vi "PathPlanner_Path_PreCalcValues.vi"(11 "PathPlannerPath":T1={"Reversed"=FALSE, "RotationTargets"=[], "ConstraintZones"=[], "EventMarkers"=[], "GlobalConstraints"={"MaxVelocityMps;"=0.0, "MaxAccelerationMpsSq;"=0.0, "MaxAngularVelRadPsEc;"=0.0, "MaxAngularAccRadPSecSq"=0.0, "Exists"=FALSE, "Unlimited"=FALSE, "NominalVoltageVolts"=12.0}, "GoalEndState"={"VelocityMPS"=0.0, "Rotation"={"VALUE"=0.0, "COS"=1.0, "SIN"=0.0}}, "AllPoints"=[], "Name"="", "Waypoints"=[], "PointTowardsZones"=[], "IdealStartingState"={"VelocityMPS"=0.0, "Rotation"={"VALUE"=1.0, "COS"=0.0, "SIN"=0.0}}, "IsChoreoPath"=FALSE, "PreventFlipping"=FALSE} {"IdealStartingState"."Rotation"."SIN" format="%13.4f"; "IdealStartingState"."Rotation"."COS" format="%13.4f"; "IdealStartingState"."Rotation"."VALUE" format="%13.4f"; "PointTowardsZones"."TargetPosition"."Y" format="%14.3f"; "PointTowardsZones"."TargetPosition"."X" format="%14.3f"; "PointTowardsZones"."RotationOffset"."SIN" format="%13.4f"; "PointTowardsZones"."RotationOffset"."COS" format="%13.4f"; "PointTowardsZones"."RotationOffset"."VALUE" format="%13.4f"; "Waypoints"."nextControl"."Y" format="%14.3f"; "Waypoints"."nextControl"."X" format="%14.3f"; "Waypoints"."anchor"."Y" format="%14.3f"; "Waypoints"."anchor"."X" format="%14.3f"; "Waypoints"."prevControl"."Y" format="%14.3f"; "Waypoints"."prevControl"."X" format="%14.3f"; "AllPoints"."RotationTarget"."rotation"."SIN" format="%13.4f"; "AllPoints"."RotationTarget"."rotation"."COS" format="%13.4f"; "AllPoints"."RotationTarget"."rotation"."VALUE" format="%13.4f"; "AllPoints"."Position"."Y" format="%14.3f"; "AllPoints"."Position"."X" format="%14.3f"; "GoalEndState"."Rotation"."SIN" format="%13.4f"; "GoalEndState"."Rotation"."COS" format="%13.4f"; "GoalEndState"."Rotation"."VALUE" format="%13.4f"; "RotationTargets"."rotation"."SIN" format="%13.4f"; "RotationTargets"."rotation"."COS" format="%13.4f"; "RotationTargets"."rotation"."VALUE" format="%13.4f"}) -> (3 "out PathPlannerPath":T1={"Reversed"=FALSE, "RotationTargets"=[], "ConstraintZones"=[], "EventMarkers"=[], "GlobalConstraints"={"MaxVelocityMps;"=0.0, "MaxAccelerationMpsSq;"=0.0, "MaxAngularVelRadPsEc;"=0.0, "MaxAngularAccRadPSecSq"=0.0, "Exists"=FALSE, "Unlimited"=FALSE, "NominalVoltageVolts"=12.0}, "GoalEndState"={"VelocityMPS"=0.0, "Rotation"={"VALUE"=0.0, "COS"=1.0, "SIN"=0.0}}, "AllPoints"=[], "Name"="", "Waypoints"=[], "PointTowardsZones"=[], "IdealStartingState"={"VelocityMPS"=0.0, "Rotation"={"VALUE"=1.0, "COS"=0.0, "SIN"=0.0}}, "IsChoreoPath"=FALSE, "PreventFlipping"=FALSE} {"IdealStartingState"."Rotation"."SIN" format="%13.4f"; "IdealStartingState"."Rotation"."COS" format="%13.4f"; "IdealStartingState"."Rotation"."VALUE" format="%13.4f"; "PointTowardsZones"."TargetPosition"."Y" format="%14.3f"; "PointTowardsZones"."TargetPosition"."X" format="%14.3f"; "PointTowardsZones"."RotationOffset"."SIN" format="%13.4f"; "PointTowardsZones"."RotationOffset"."COS" format="%13.4f"; "PointTowardsZones"."RotationOffset"."VALUE" format="%13.4f"; "Waypoints"."nextControl"."Y" format="%14.3f"; "Waypoints"."nextControl"."X" format="%14.3f"; "Waypoints"."anchor"."Y" format="%14.3f"; "Waypoints"."anchor"."X" format="%14.3f"; "Waypoints"."prevControl"."Y" format="%14.3f"; "Waypoints"."prevControl"."X" format="%14.3f"; "AllPoints"."RotationTarget"."rotation"."SIN" format="%13.4f"; "AllPoints"."RotationTarget"."rotation"."COS" format="%13.4f"; "AllPoints"."RotationTarget"."rotation"."VALUE" format="%13.4f"; "AllPoints"."Position"."Y" format="%14.3f"; "AllPoints"."Position"."X" format="%14.3f"; "GoalEndState"."Rotation"."SIN" format="%13.4f"; "GoalEndState"."Rotation"."COS" format="%13.4f"; "GoalEndState"."Rotation"."VALUE" format="%13.4f"; "RotationTargets"."rotation"."SIN" format="%13.4f"; "RotationTargets"."rotation"."COS" format="%13.4f"; "RotationTargets"."rotation"."VALUE" format="%13.4f"})   [LabVIEW 2019, in "PathPlanner24.lvlib"]
doc: "This is an internal routine.\n\nInputs: \n - Path - cluster - path definition data structure\n\nOutputs:\n - Path - cluster - path definition data structure"
uses:
  PathPlanner24.lvlib
  <vilib>/Rock Robotics/WPI/ThirdParty/JAS_Junk/TrajLib/Trajectory_Library.lvlib
  <vilib>/Rock Robotics/WPI/ThirdParty/JAS_Junk/TrajLib/TypeDef/TRANSLATION2D.ctl
  <vilib>/Rock Robotics/WPI/ThirdParty/JAS_Junk/TrajLib/TypeDef/ROTATION2D.ctl
  TypeDef/PathPlannerPathConstraints.ctl
  TypeDef/PathPlannerRotationTarget.ctl
  TypeDef/PathPlannerConstraintsZone.ctl
  TypeDef/PathPlannerEventMarker.ctl
  TypeDef/PathPlannerGoalEndState.ctl
  TypeDef/PathPlannerPathPoint.ctl
  TypeDef/PathPlannerPath.ctl
  TypeDef/PathPlannerCommandUtil.ctl
  ENum/PathPlanner_TrajectoryEvent_Type_ENUM.ctl
  TypeDef/PathPlannerWaypoint.ctl
  TypeDef/PathPlannerPointTowardsZone.ctl
  TypeDef/PathPlannerIdealStartingState.ctl
  ENum/PathPlanner_CommandUtil_Type_ENUM.ctl
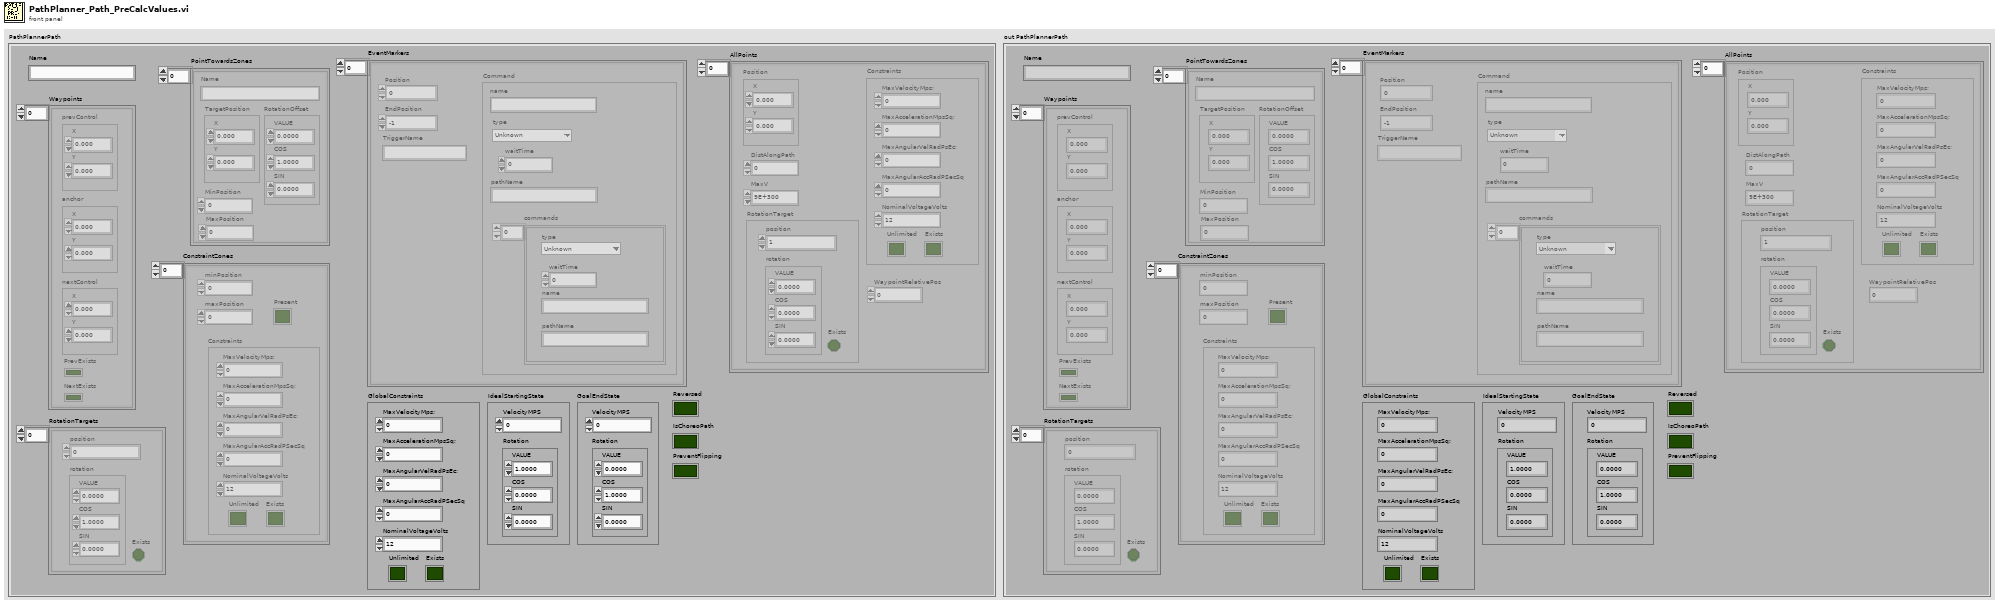
[diagram p1: front panel]
types:
  T1 = typedef "PathPlanner24.lvlib/PathPlannerPath.ctl" = cluster{"Reversed":bool, "RotationTargets":T2[], "ConstraintZones":T4[], "EventMarkers":T6[], "GlobalConstraints":T5, "GoalEndState":T10, "AllPoints":T11[], "Name":string, "Waypoints":T13[], "PointTowardsZones":T14[], "IdealStartingState":T15, "IsChoreoPath":bool, "PreventFlipping":bool}
  T2 = typedef "PathPlanner24.lvlib/PathPlannerRotationTarget.ctl" = cluster{"position":dbl, "rotation":T3, "Exists":bool}
  T3 = typedef "Trajectory_Library.lvlib/ROTATION2D.ctl" = cluster{"VALUE":dbl, "COS":dbl, "SIN":dbl}
  T4 = typedef "PathPlanner24.lvlib/PathPlannerConstraintsZone.ctl" = cluster{"minPosition":dbl, "maxPosition":dbl, "Constraints":T5, "Present":bool}
  T5 = typedef "PathPlanner24.lvlib/PathPlannerPathConstraints.ctl" = cluster{"MaxVelocityMps;":dbl, "MaxAccelerationMpsSq;":dbl, "MaxAngularVelRadPsEc;":dbl, "MaxAngularAccRadPSecSq":dbl, "Exists":bool, "Unlimited":bool, "NominalVoltageVolts":dbl}
  T6 = typedef "PathPlanner24.lvlib/PathPlannerEventMarker.ctl" = cluster{"Position":dbl, "Command":T7, "TriggerName":string, "EndPosition":dbl}
  T7 = typedef "PathPlanner24.lvlib/PathPlannerCommandUtil.ctl" = cluster{"waitTime":dbl, "name":string, "pathName":string, "commands":cluster{"type":T8, "waitTime":dbl, "name":string, "pathName":string}[], "type":T9}
  T8 = typedef "PathPlanner24.lvlib/PathPlanner_TrajectoryEvent_Type_ENUM.ctl" = enum16{"Unknown", "Wait", "Named", "Path", "Sequential", "Parallel", "Race", "Deadline", "PointTowardsZoneEnter", "PointTowardsZoneExit", "TriggerEventStart", "TriggerEventStop", "TriggerEventOneshot"}
  T9 = typedef "PathPlanner24.lvlib/PathPlanner_CommandUtil_Type_ENUM.ctl" = enum16{"Unknown", "Wait", "Named", "Path", "Sequential", "Parallel", "Race", "Deadline"}
  T10 = typedef "PathPlanner24.lvlib/PathPlannerGoalEndState.ctl" = cluster{"VelocityMPS":dbl, "Rotation":T3}
  T11 = typedef "PathPlanner24.lvlib/PathPlannerPathPoint.ctl" = cluster{"Position":T12, "DistAlongPath":dbl, "MaxV":dbl, "Constraints":T5, "RotationTarget":T2, "WaypointRelativePos":dbl}
  T12 = typedef "Trajectory_Library.lvlib/TRANSLATION2D.ctl" = cluster{"X":dbl, "Y":dbl}
  T13 = typedef "PathPlanner24.lvlib/PathPlannerWaypoint.ctl" = cluster{"prevControl":T12, "anchor":T12, "nextControl":T12, "PrevExists":bool, "NextExists":bool}
  T14 = typedef "PathPlanner24.lvlib/PathPlannerPointTowardsZone.ctl" = cluster{"RotationOffset":T3, "Name":string, "TargetPosition":T12, "MinPosition":dbl, "MaxPosition":dbl}
  T15 = typedef "PathPlanner24.lvlib/PathPlannerIdealStartingState.ctl" = cluster{"VelocityMPS":dbl, "Rotation":T3}
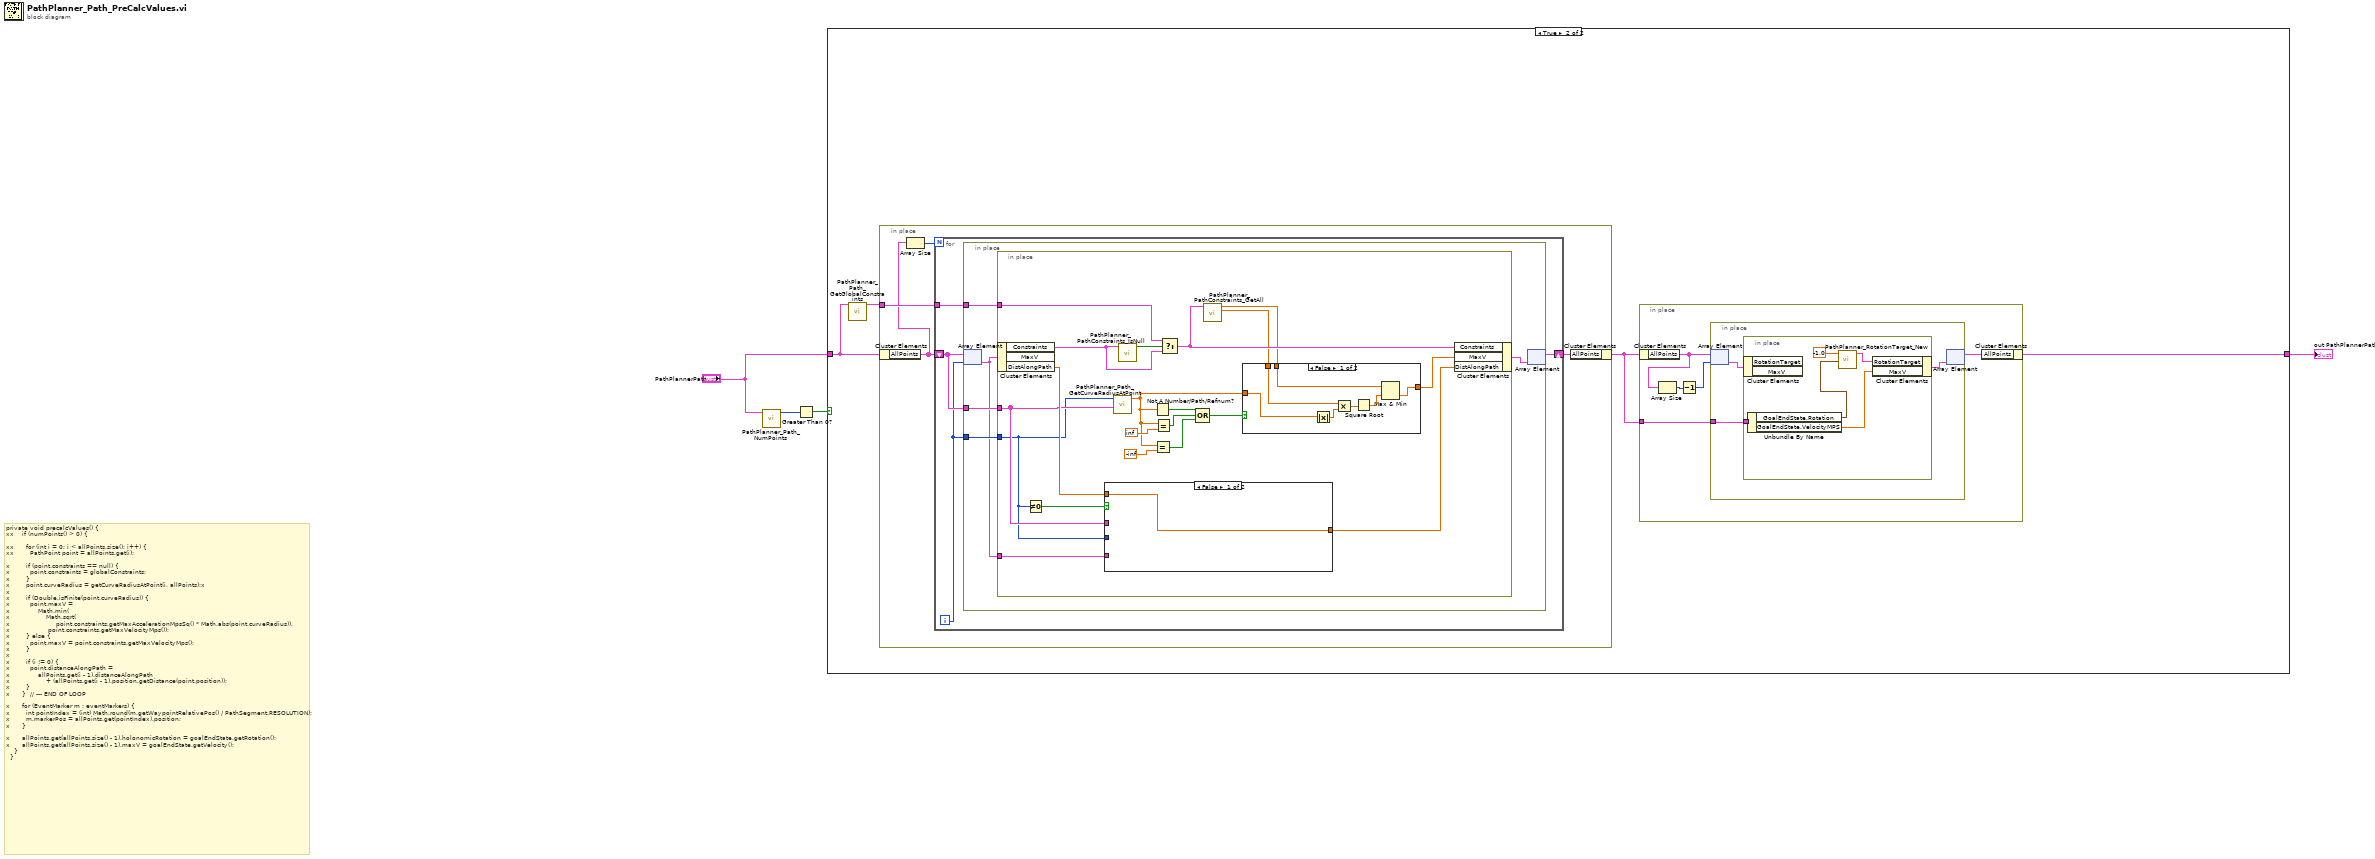
[diagram p0: block diagram]
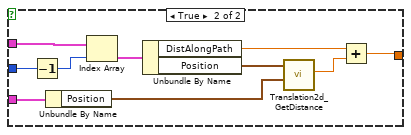
[diagram p3: hidden frame]
diagram:
  # "private void precalcValues() {\nxx    if (numPoints() > 0) {\n\nxx      for (int i = 0; i < allPoints.size(); i++) {\nxx        PathPoint point = allPoints.get(i);\n\nx        if (point.constraints == null) {\nx          point.constraints = globalConstraints;\nx        }\nx        point.curveRadius = getCurveRadiusAtPoint(i, allPoints);x\nx\nx        if (Double.isFinite(point.curveRadius)) {\nx          point.maxV =\nx              Math.min(\nx                  Math.sqrt(\nx                      \tpoint.constraints.getMaxAccelerationMpsSq() * Math.abs(point.curveRadius)),\nx                  \tpoint.constraints.getMaxVelocityMps());\nx        } else {\nx          point.maxV = point.constraints.getMaxVelocityMps();\nx        }\nx\nx        if (i != 0) {\nx          point.distanceAlongPath =\nx              allPoints.get(i - 1).distanceAlongPath\nx                  + (allPoints.get(i - 1).position.getDistance(point.position));\nx        }\nx      }  // --- END OF LOOP\n\nx      for (EventMarker m : eventMarkers) {\nx        int pointIndex = (int) Math.round(m.getWaypointRelativePos() / PathSegment.RESOLUTION);\nx        m.markerPos = allPoints.get(pointIndex).position;\nx      }\n\nx      allPoints.get(allPoints.size() - 1).holonomicRotation = goalEndState.getRotation();\nx      allPoints.get(allPoints.size() - 1).maxV = goalEndState.getVelocity();\n    }\n  }"
  n1 = call "PathPlanner_Path_NumPoints.vi"("PathPlannerPath"="PathPlannerPath") -> ("NumPoints"=w4:i32)  [unwired: 10 in]
  n2 = Greater Than 0?(x=w4) -> (x > 0?=w3:bool)
  n3 = case shown="True" w3 {
    tunnel: "PathPlannerPath" -> [w5 w6]
    tunnel: [w5 w9] -> w2
    frame False {
    }
    frame True {
      n4 = call "PathPlanner_Path_GetGlobalConstraints.vi"("PathPlannerPath"=w6) -> ("GlobalConstraints"=w7:T5)  [unwired: 10 in]
      n5 = in-place {
        in-place-border: w7 -> [w26]
        n6 = in-place-cluster #1(w6) -> ("AllPoints"=w24:T11[])
        n7 = Array Size(array=w24) -> (size(s)=w25:i32)
        n8 = for {
          N: w25 -> [_]
          tunnel: w26 -> [w30]
          shift-right: [w27] -> w23
          shift-left: w24 -> [w29]
          i -> [w28]
          n9 = in-place {
            in-place-border: w30 -> [w34]
            in-place-border: w29 -> [w33]
            in-place-border: w28 -> [w32]
            n10 = in-place-array #2(w29, w28) -> (w31:T11)
            n11 = in-place {
              in-place-border: w34 -> [w53]
              in-place-border: w33 -> [w41]
              in-place-border: w32 -> [w40]
              in-place-border: w31 -> [w39]
              n12 = in-place-cluster #3(w31) -> ("Constraints"=w54:T5, "DistAlongPath"=w43:dbl)  [unwired: 1 out]
              n13 = Not Equal To 0?(x=w40) -> (x != 0?=w44:bool)
              n14 = case shown="False" w44 {
                tunnel: w43 -> [w56 _]
                tunnel: [w56 w57] -> w42
                tunnel: w41 -> [_ w66]
                tunnel: w40 -> [_ w64]
                tunnel: w39 -> [_ w61]
                frame False {
                }
                frame True {
                  n15 = Decrement(x=w64) -> (x-1=w65:i32)
                  n16 = Unbundle By Name(w61) -> ("Position"=w60:T12)
                  n17 = Index Array(array=w66, index=w65) -> (element=w63:T11)
                  n18 = Unbundle By Name(w63) -> ("DistAlongPath"=w59:dbl, "Position"=w62:T12)
                  n19 = call <vilib>:"Translation2d_GetDistance.vi"("other Translation"=w60, "In Translation"=w62) -> ("Distance"=w58:dbl)  [unwired: 9 in]
                  n20 = Add(x=w59, y=w58) -> (x+y=w57:dbl)
                }
              }
              n21 = call "PathPlanner_Path_GetCurveRadiusAtPoint.vi"("Points"=w41, "Index"=w40) -> ("Radius"=w36:dbl)  [unwired: 9 in]
              n22 = call "PathPlanner_PathConstraints_IsNull.vi"("PathPlannerConstraints"=w54) -> ("IsNull"=w55:bool)  [unwired: 10 in]
              n23 = Not A Number/Path/Refnum?(number/path/refnum=w36) -> (NaN/Path/Refnum?=w49:bool)
              n24 = Equal?(x=w36, y=-inf) -> (x = y?=w37:bool)
              n25 = Equal?(x=w36, y=inf) -> (x = y?=w48:bool)
              n26 = Select(t=w53, s=w55, f=w54) -> (s? t:f=w52:T5)
              n27 = Compound Arithmetic op=OR(w49, w48, w37) -> (w46:bool)
              n28 = call "PathPlanner_PathConstraints_GetAll.vi"("PathPlannerConstraints"=w52) -> ("MaxAccelerationMpsSq;"=w45:dbl, "MaxVelocityMps;"=w51:dbl)  [unwired: 6 in, 3 out]
              n29 = case shown="False" w46 {
                tunnel: w51 -> [w72 w74]
                tunnel: [w73 w74] -> w50
                tunnel: w45 -> [w69 _]
                tunnel: w36 -> [w67 _]
                frame False {
                  n30 = Absolute Value(x=w67) -> (abs(x)=w70:dbl)
                  n31 = Multiply(x=w69, y=w70) -> (x*y=w68:dbl)
                  n32 = Square Root(x=w68) -> (sqrt(x)=w71:dbl)
                  n33 = Max & Min(x=w72, y=w71) -> (min(x,y)=w73:dbl)  [unwired: 1 out]
                }
                frame True {
                }
              }
              n34 = in-place-cluster #3("Constraints"=w52, "MaxV"=w50, "DistAlongPath"=w42) -> (w35:T11)
            }
            n35 = in-place-array #2(w35) -> (w27:T11[])  [unwired: 1 out]
          }
        }
        n36 = in-place-cluster #1("AllPoints"=w23) -> (w8:T1)
      }
      n37 = in-place {
        in-place-border: w8 -> [w10]
        n38 = in-place-cluster #4(w8) -> ("AllPoints"=w13:T11[])
        n39 = Array Size(array=w13) -> (size(s)=w14:i32)
        n40 = Decrement(x=w14) -> (x-1=w12:i32)
        n41 = in-place {
          in-place-border: w10 -> [w15]
          n42 = in-place-array #5(w13, w12) -> (w17:T11)
          n43 = in-place {
            in-place-border: w15 -> [w22]
            n44 = in-place-cluster #6(w17) -> ()  [unwired: 2 out]
            n45 = Unbundle By Name(w22) -> ("GoalEndState.Rotation"=w19:T3, "GoalEndState.VelocityMPS"=w21:dbl)
            n46 = call "PathPlanner_RotationTarget_New.vi"("rotation"=w19, "position"=-1.0) -> ("RotationTarget"=w18:T2)  [unwired: 9 in]
            n47 = in-place-cluster #6("RotationTarget"=w18, "MaxV"=w21) -> (w16:T11)
          }
          n48 = in-place-array #5(w16) -> (w11:T11[])  [unwired: 1 out]
        }
        n49 = in-place-cluster #4("AllPoints"=w11) -> (w9:T1)
      }
    }
  }
  "out PathPlannerPath" <- w2
